vi "CSM - Mark As Chain Module.vi"(6 "Order":i32, 9 "CSM Name":string="Chain") -> (2 "CSM Name (Marked As Chain)":string)   [LabVIEW 2017, in "Communicable State Machine.lvlib"]
doc: "Concatenates the name of a Chain of Responsibility Mode module, using `$` as the separator. Note that the order does not need to be consecutive, but it must be unique. Nodes with smaller numbers are arranged at the front of the responsibility chain.\n\n<b>Reference Example</b>: `4. Advance Examples\\2. Chain of Responsibility Example`.\n\n\n> [!NOTE] <b>CSM Chain of Responsibility Mode</b>\n>\n> Multiple CSM modules form a complete module via Chain of Responsibility Mode by appending `$` to the requested name to form a chain for processing transactions.\n> - From an external call perspective, these instances collectively form a composite module named Chain.\n> - Each instance is named a Chain Node.\n>\n> <b>Behavior</b>: External callers can consider the Chain as a single CSM module capable of message communication, state registration, and so on. Internally, nodes attempt to process the message sequentially according to their order. When a node has the capability to process the current message, the message is processed and is not passed further down the chain.\n>\n> <b>Example</b>:\n>\n> // Request module name as `module$`, where `module` is the chain name. Instantiate 4 instances. Their names might be:\n> // - `module$1`\n> // - `module$2`\n> // - `module$3`\n> // - `module$4`\n> // The sequence of the composed Chain is `module$1(head) >> module$2 >> module$3 >> module$4(tail)`\n> // Assume `module$3` and `module$4` can process \"csm message\"\n> `csm message >> arguments -@ module`\n> // This message will be processed by `module$3`. `module$4` will not respond.\n>\n> <b>Application Scenarios</b>:\n> - Permission approval process. Based on job hierarchy, personnel with specific functional permissions can approve directly without passing it further.\n> - Function concatenation. Different modules implement different tasks, and different functional sets can be combined through concatenation.\n> - Function overriding. Implementing overloading in OOP through overriding.\n> - Worker Mode scenarios are usually not suitable for having UI operations.\n\n\n> [!NOTE] <b>Name Concatenation API</b>\n>\n> This VI only manipulates the module name string and has no actual functionality. Therefore, once you are familiar with the CSM rules, you can directly enter name string and rule symbols without calling this API.\n\n\n-- <b>Controls</b> --\n- <b>CSM Name</b>: CSM module name.\n- <b>Order</b>: Sequence in Chain of Responsibility Mode. Nodes with smaller numbers are arranged at the front of the responsibility chain.\n\n-- <b>Indicators</b> --\n- <b>CSM Name (Marked As Chain)</b>: CSM module name marked with `$`."
uses:
  Communicable State Machine.lvlib
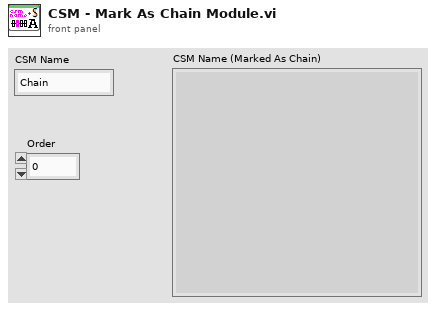
[diagram p1: front panel]
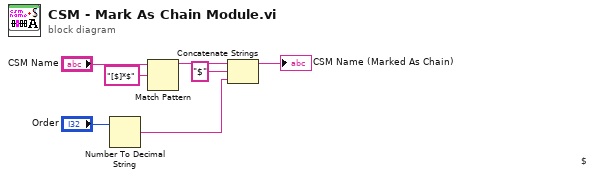
[diagram p0: block diagram]
diagram:
  # "$"
  n1 = Number To Decimal String(number="Order") -> (decimal integer string=w1:string)  [unwired: 1 in]
  n2 = Match Pattern(string="CSM Name", regular expression="[$]*$") -> (before substring=w5:string)  [unwired: 1 in, 3 out]
  n3 = Concatenate Strings(w5, "$" ("string"), w1) -> (→"CSM Name (Marked As Chain)":string)
